vi "MetaData Channel.vi"(8 "error in (no error)":errorcluster, 11 "Node Ptr":T5 format="%.0x") -> (0 "error out":errorcluster)   [LabVIEW 2020, in "Instrument Addon System Explorer.lvlib"]
uses:
  Instrument Addon System Explorer.lvlib
  <vilib>/NI VeriStand/Custom Device API/Custom Device API.lvlib
  Addon Shared/Instrument Addon Shared.lvlib
  Addon Shared/Types/FG Control.ctl
  Addon Shared/SubVIs/Constants.vi
  APIs/Scripting API/Instrument Addon Scripting API.lvlib
  <vilib>/NI VeriStand/Custom Device API/Custom Device Item Ref.ctl
  Addon Shared/Types/Protocol Data Type.ctl
  Addon Shared/Types/Metadata Channel Type.ctl
  Addon Shared/Types/Type Cast Type.ctl
  Addon Shared/Types/Endian.ctl
panel:
  in  "Delimiter":string=","
  in  "Reset":bool
  in  "Create":bool
  in  "Elements":u32
  in  "Units":string
  in  "Default Value":dbl
  out "Channel Type (Tab)":enum32{"List", "Format", "Type Cast"}(tab)
  in  "Remove":bool
  in  "Add":bool
  in  "Enumerated List":i32(listbox)
  in  "Test Value":dbl
  in  "Format String":string="%.3g"
  out "Validated String":string
  in  "Endian":T1=enum."Little"
  in  "Type":T2
  in  "Channel Type":T3
  out "Data Type":T4
  in  "Header 2":cluster{"Section Name":string}={"Section Name"="MetaData Format Settings"}
  in  "SHDocVw.IWebBrowser":refnum<k7>(container)
  in  "Header":cluster{"Section Name":string}={"Section Name"="MetaData Settings"}
  in  "Description":string
  in  "Name":string
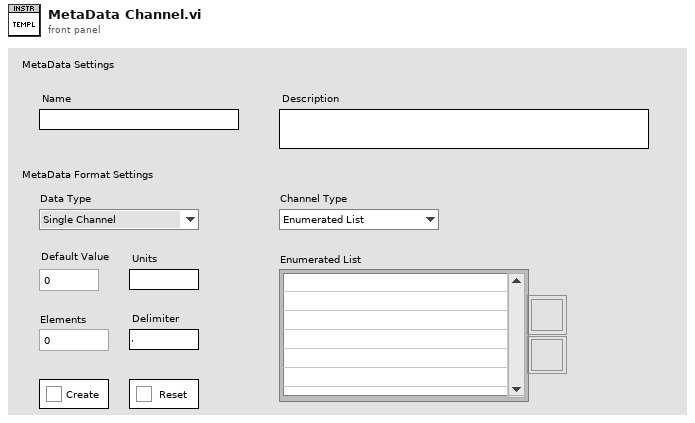
[diagram p1: front panel]
types:
  T1 = typedef "Instrument Addon Shared.lvlib/Endian.ctl" = enum16{"Native", "Little", "Big"}
  T2 = typedef "Instrument Addon Shared.lvlib/Type Cast Type.ctl" = enum16{"DBL", "SGL", "U64", "U32", "U16", "U8", "I64", "I32", "I16", "I8"}
  T3 = typedef "Instrument Addon Shared.lvlib/Metadata Channel Type.ctl" = enum16{"Enumerated List", "Format", "Type Cast"}
  T4 = typedef "Instrument Addon Shared.lvlib/Protocol Data Type.ctl" = enum16{"Single Channel", "Array"}
  T5 = typedef "Custom Device API.lvlib/Custom Device Item Ref.ctl" = u64
  T6 = typedef "Instrument Addon Shared.lvlib/FG Control.ctl" = enum16{"Get", "Set"}
  T7 = typedef "Custom Device API.lvlib/Custom Device Item Info.ctl" = cluster{"Name":string, "Is Channel":bool, "GUID":string, "Is Waveform":bool}
  T8 = typedef "Instrument Addon Shared.lvlib/MetaData Parameters.ctl" = cluster{"Data Type":T4, "Channel Type":T3, "List":string[], "Format String":string, "Type":T2, "Delimiter":string, "Endian":T1}
  T9 = typedef "Custom Device API.lvlib/Custom Device Channel.ctl" = cluster{"Type":T10, "Units":string, "Default Value":dbl, "Faultable":bool, "Scalable":bool}
  T10 = typedef "Custom Device API.lvlib/Custom Device Channel Type.ctl" = enum16{"Input", "Output"}
  T11 = typedef "Custom Device API.lvlib/Custom Device Commands.ctl" = enum16{"Default", "Item renamed", "Shutdown", "Dynamic button pressed"}
  T12 = typedef "Instrument Addon Scripting API.lvlib/Array Element.ctl" = cluster{"Name":string, "Default Value":dbl, "Units":string}
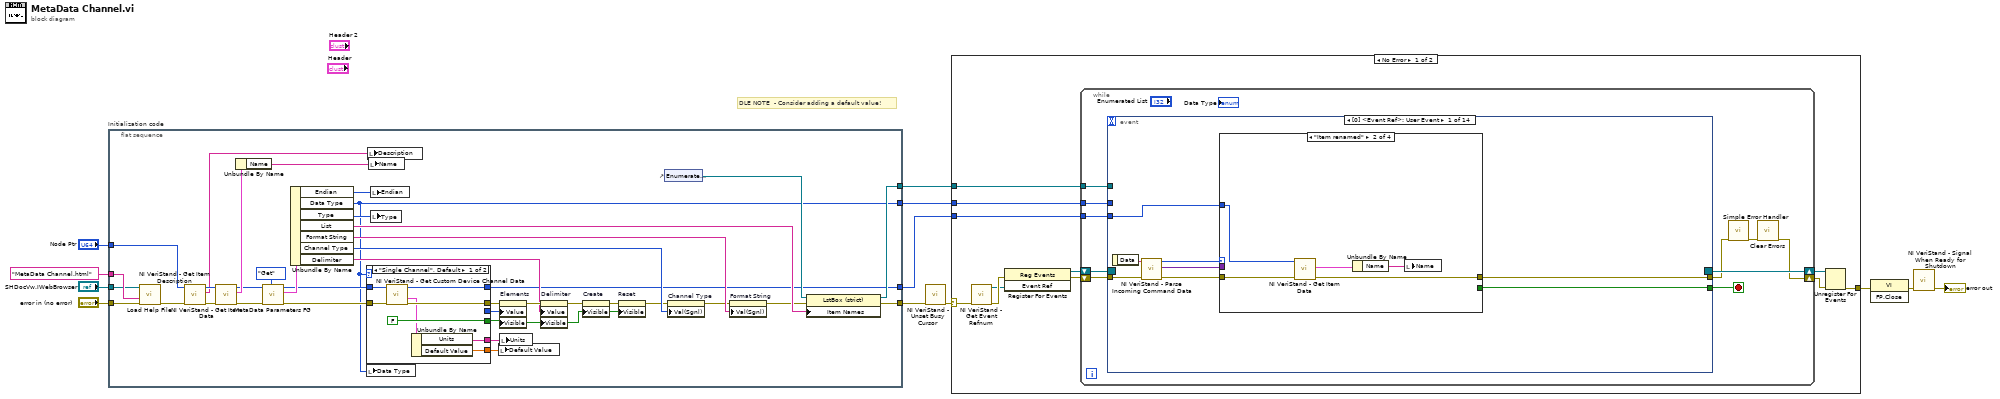
[diagram p0: block diagram]
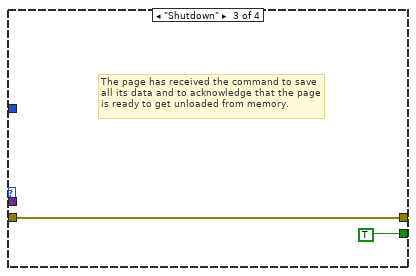
[diagram p3: hidden frame]
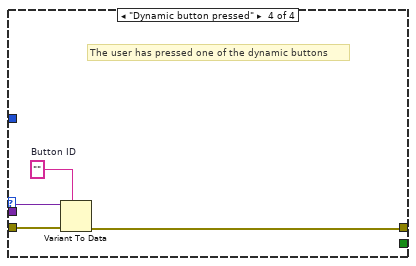
[diagram p4: hidden frame]
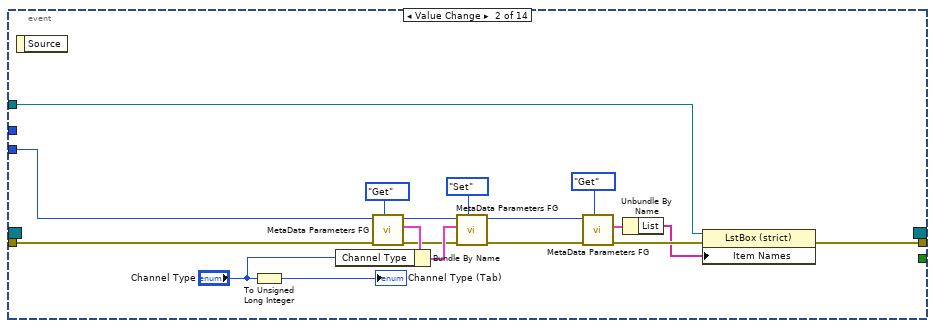
[diagram p5: hidden frame]
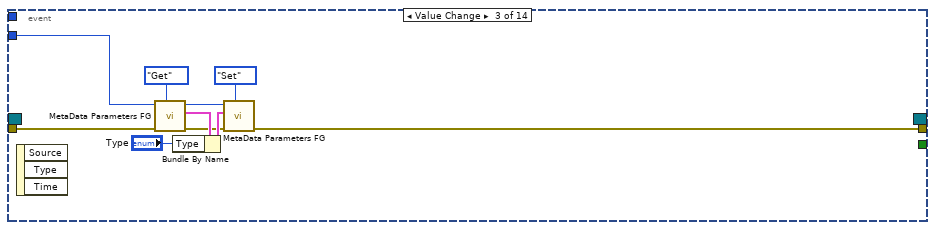
[diagram p6: hidden frame]
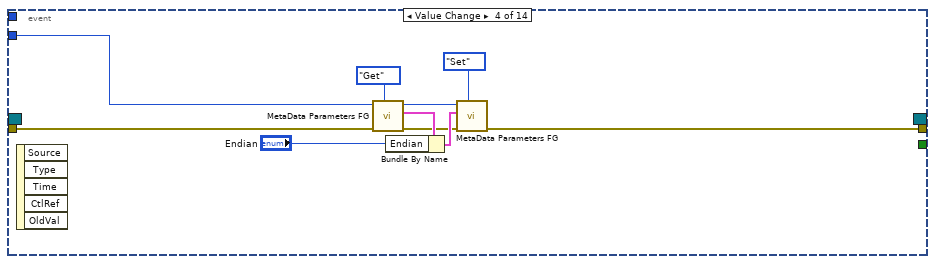
[diagram p7: hidden frame]
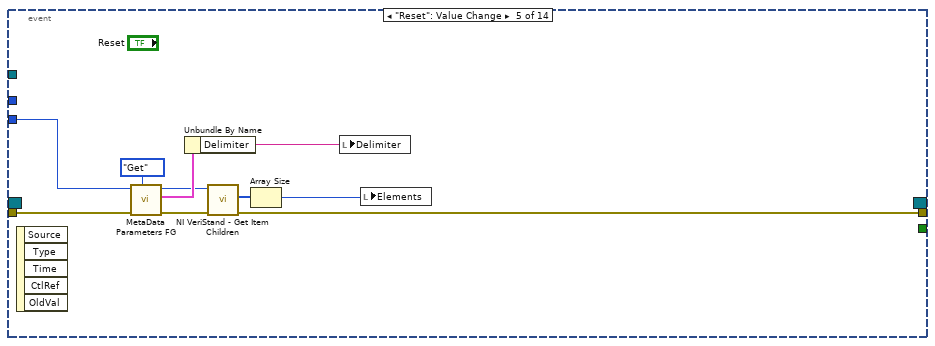
[diagram p8: hidden frame]
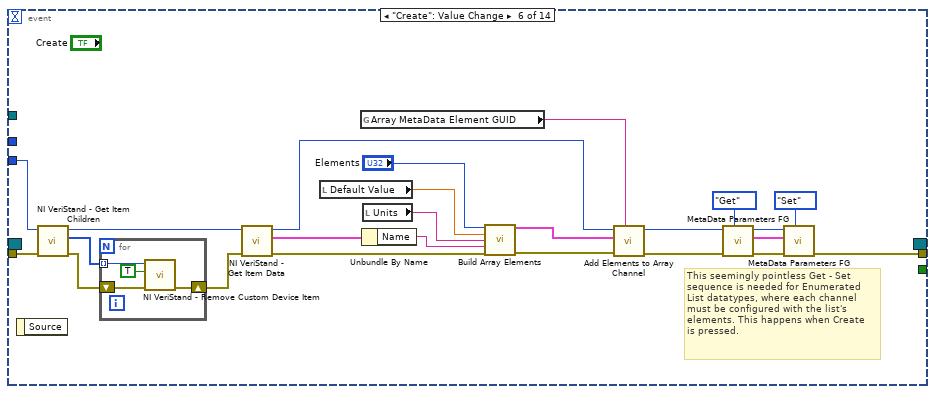
[diagram p9: hidden frame]
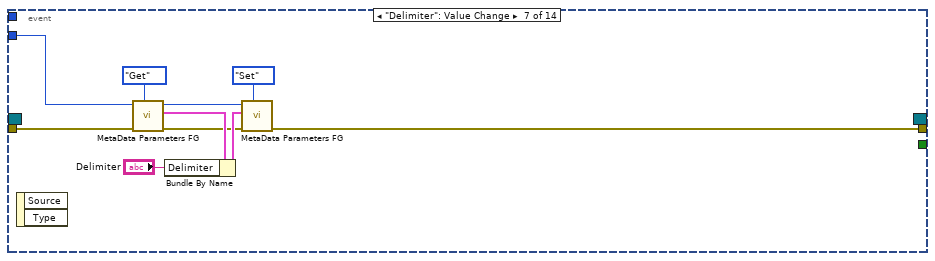
[diagram p10: hidden frame]
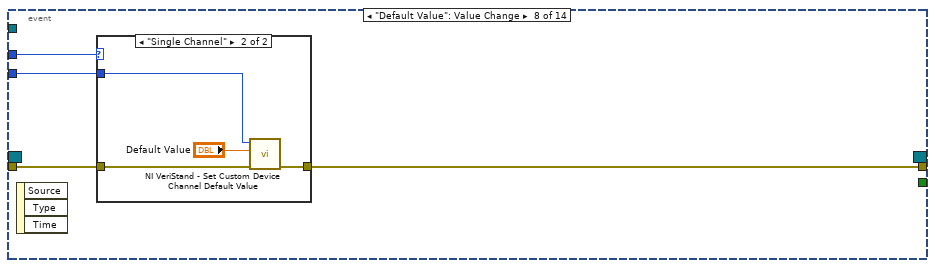
[diagram p11: hidden frame]
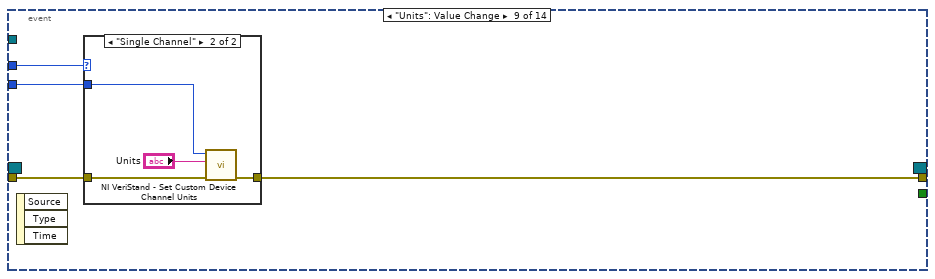
[diagram p13: hidden frame]
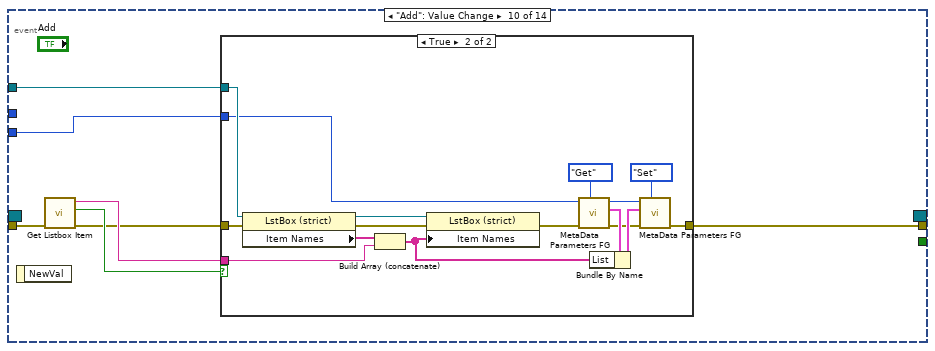
[diagram p15: hidden frame]
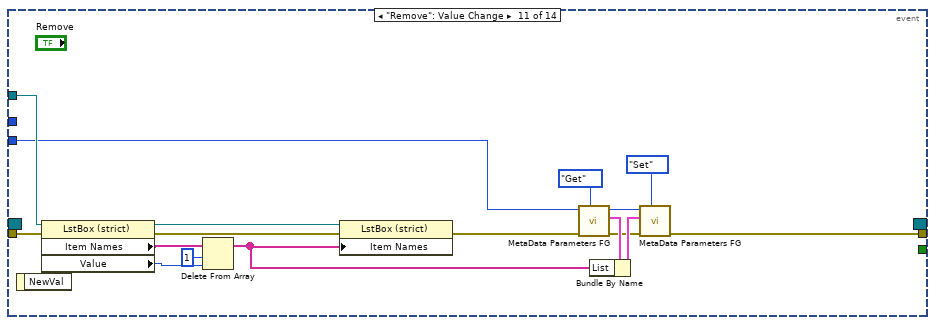
[diagram p17: hidden frame]
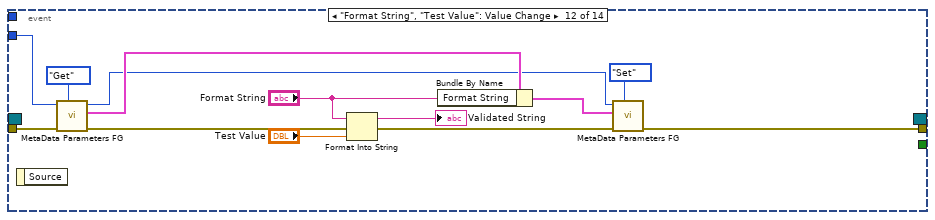
[diagram p18: hidden frame]
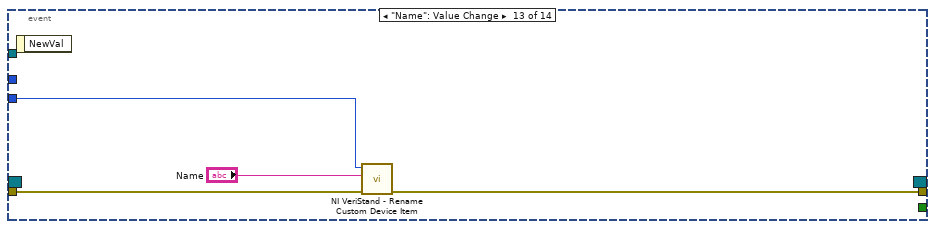
[diagram p19: hidden frame]
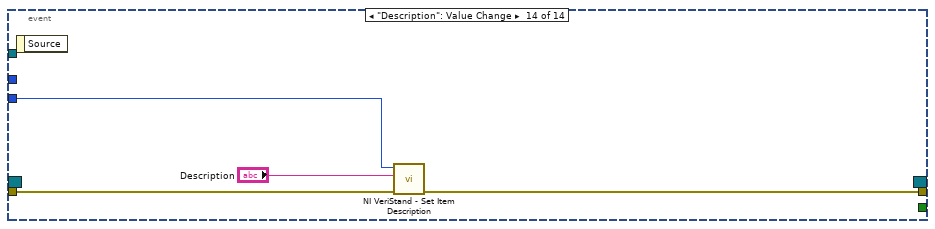
[diagram p20: hidden frame]
diagram:
  # "DLE NOTE  - Consider adding a default value!"
  n1 = flat-sequence "Initialization code" {
    tunnel: "error in (no error)" -> [w45]
    tunnel: "Node Ptr" -> [w31]
    tunnel: [w35] -> w8
    tunnel: [w19] -> w2
    tunnel: "MetaData Channel.html" ("HTML File") -> [w44]
    tunnel: "SHDocVw.IWebBrowser" -> [w43]
    tunnel: [w33] -> w3
    tunnel: [w16] -> w1
    frame #0 {
      n2 = call "Load Help File.vi"("error in (no error)"=w45, "HTML File to Load"=w44, "SHDocVw.IWebBrowser2"=w43) -> ("error out"=w32:errorcluster)  [unwired: 8 in]
      n3 = call <vilib>:"NI VeriStand - Get Item Description.vi"("error in (no error)"=w32, "Item Ref in"=w31) -> ("error out"=w48:errorcluster, "Description"=w49:string, "Item Ref out"=w50:T5)  [unwired: 7 out]
      n4 = call <vilib>:"NI VeriStand - Get Item Data.vi"("error in (no error)"=w48, "Item Ref in"=w50) -> ("error out"=w24:errorcluster, "Item Info"=w47:T7, "Item Ref out"=w23:T5)  [unwired: 7 out]
      n5 = Unbundle By Name(w47) -> ("Name"=w46:string)
      n6 = call "MetaData Parameters FG.vi"("Action"=FG_Control."Get", "error in (no error)"=w24, "Item Ref in"=w23) -> ("error out"=w22:errorcluster, "MetaData Parameters"=w41:T8, "Item Ref out"=w21:T5)  [unwired: 6 in]
      n7 = Unbundle By Name(w41) -> ("Endian"=w14:T1, "Data Type"=w16:T4, "Type"=w30:T2, "List"=w39:string[], "Format String"=w38:string, "Channel Type"=w40:T3, "Delimiter"=w25:string)
      n8 = local write "Data Type"(w16) -> ()
      n9 = case shown="\"Single Channel\", Default" w16 {
        tunnel: [FALSE TRUE] -> w13
        tunnel: w22 -> [w57 w62]
        tunnel: w21 -> [w56 w66]
        tunnel: [w55 w61] -> w20
        tunnel: [w54 w63] -> w19
        tunnel: [w52 ""] -> w18
        tunnel: [w51 0.0 ("Default Value")] -> w17
        tunnel: [_ w59] -> w15
        frame "Single Channel", Default {
          n10 = call <vilib>:"NI VeriStand - Get Custom Device Channel Data.vi"("error in (no error)"=w57, "Channel Ref in"=w56) -> ("error out"=w55:errorcluster, "Channel"=w53:T9, "Channel Ref out"=w54:T5)  [unwired: 4 in, 3 out]
          n11 = Unbundle By Name(w53) -> ("Units"=w52:string, "Default Value"=w51:dbl)
        }
        frame "Array" {
          n12 = call <vilib>:"NI VeriStand - Get Item Children.vi"("error in (no error)"=w62, "Item Ref in"=w66) -> ("error out"=w61:errorcluster, "Child Refs"=w60:T5[], "Item Ref out"=w63:T5)  [unwired: 6 in, 1 out]
          n13 = Array Size(array=w60) -> (size(s)=w59:i32)
        }
      }
      n14 = local write "Description"(w49) -> ()
      n15 = local write "Name"(w46) -> ()
      n16 = local write "Endian"(w14) -> ()
      n17 = local write "Type"(w30) -> ()
      n18 = local write "Default Value"(w17) -> ()
      n19 = property on="Elements" class="DigNum (strict)"(error in=w20, "Value"=w15, "Visible"=w13) -> (error out=w27:errorcluster)  [unwired: 1 in, 1 out]
      n20 = local write "Units"(w18) -> ()
      n21 = property on="Delimiter" class="Str"(error in=w27, "Value"=w25, "Visible"=w13) -> (error out=w28:errorcluster)  [unwired: 1 in, 1 out]
      n22 = property on="Create" class="Bool"(error in=w28, "Visible"=w13) -> (error out=w29:errorcluster)  [unwired: 1 in, 1 out]
      n23 = property on="Reset" class="Bool"(error in=w29, "Visible"=w13) -> (error out=w26:errorcluster)  [unwired: 1 in, 1 out]
      n24 = control-ref of="Enumerated List"() -> (w34:refnum<vi>)
      n25 = property on="Channel Type" class="Enum (strict)"(error in=w26, "Val(Sgnl)"=w40) -> (error out=w37:errorcluster)  [unwired: 1 in, 1 out]
      n26 = property on="Format String" class="Str"(error in=w37, "Val(Sgnl)"=w38) -> (error out=w36:errorcluster)  [unwired: 1 in, 1 out]
      n27 = property class="LstBox (strict)"(reference=w34, error in=w36, "Item Names"=w39) -> (reference out=w33:refnum<vi>, error out=w35:errorcluster)
    }
  }
  n28 = call <vilib>:"NI VeriStand - Unset Busy Cursor.vi"("error in (no error)"=w8) -> ("error out"=w7:errorcluster)  [unwired: 10 out]
  n29 = case shown="No Error" w7 {
    selector: w7 -> [w70 w277]
    tunnel: [w75 w275] -> w12
    tunnel: w2 -> [w71 _]
    tunnel: w3 -> [w69 _]
    tunnel: w1 -> [w68 _]
    frame No Error {
      n30 = call <vilib>:"NI VeriStand - Get Event Refnum.vi"("error in (no error)"=w70) -> ("error out"=w78:errorcluster, "Event Ref"=w74:refnum<user-event>)  [unwired: 9 out]
      n31 = register-events(error in=w78, w74) -> (reference out=w72:refnum<event-registration>, error out=w73:errorcluster)  [unwired: 1 in]
      n32 = while {
        tunnel: w71 -> [w84]
        shift-right: [w81] -> w76
        shift-left: w73 -> [w87]
        shift-right: [w88] -> w77
        shift-left: w72 -> [w86]
        tunnel: w69 -> [w80]
        tunnel: w68 -> [w79]
        stop <- w85 stop-if-true
        n33 = event shown="[0] <Event Ref>: User Event" {
          selector: w86 -> [_ _ _ _ _ _ _ _ _ _ _ _ _ _]
          dyn-events: [_ _ _ _ _ _ _ _ _ _ _ _ _ _] -> w88
          timeout: _ -> [_ _ _ _ _ _ _ _ _ _ _ _ _ _]
          tunnel: w87 -> [w96 w120 w131 w141 w154 w176 w187 w198 w207 w214 w250 w262 w270 w273]
          tunnel: [w92 _ _ _ _ _ _ _ _ _ _ _ _ _] -> w85
          tunnel: [w91 w109 w127 w138 w148 w167 w185 w197 w206 w218 w239 w263 w269 w272] -> w83
          tunnel: w84 -> [w90 w119 w130 w140 w153 w179 w186 w196 w205 w217 w237 w260 w268 w274]
          tunnel: w80 -> [_ w111 _ _ _ _ _ _ _ w219 w253 _ _ _]
          tunnel: w79 -> [_ _ _ _ _ _ _ w195 w204 _ _ _ _ _]
          event User Event {
            n34 = event-data() -> ("Data"=w95:string)  [unwired: 1 out]
            n35 = call <vilib>:"NI VeriStand - Parse Incoming Command Data.vi"("error in (no error)"=w96, "Incoming data"=w95) -> ("error out"=w94:errorcluster, "Outgoing data"=w89:variant, "Action"=w93:T11)  [unwired: 7 out]
            n36 = case shown="\"Item renamed\"" w93 {
              tunnel: w94 -> [w97 w102 w103 w108]
              tunnel: [_ _ TRUE _] -> w92
              tunnel: [w97 w99 w103 w105] -> w91
              tunnel: w90 -> [_ w101 _ _]
              tunnel: w89 -> [_ _ _ w107]
              frame "Default", Default {
              }
              frame "Item renamed" {
                n37 = call <vilib>:"NI VeriStand - Get Item Data.vi"("error in (no error)"=w102, "Item Ref in"=w101) -> ("error out"=w99:errorcluster, "Item Info"=w100:T7)  [unwired: 8 out]
                n38 = Unbundle By Name(w100) -> ("Name"=w98:string)
                n39 = local write "Name"(w98) -> ()
              }
              frame "Shutdown" {
                # "The page has received the command to save all its data and to acknowledge that the page is ready to get unloaded from memory."
              }
              frame "Dynamic button pressed" {
                w106 = ""  # Button ID
                # "The user has pressed one of the dynamic buttons"
                n40 = Variant To Data(error in=w108, type=w106, Variant=w107) -> (error out=w105:errorcluster)  [unwired: 1 out]
              }
            }
          }
          event Value Change {
            n41 = event-data() -> ()  [unwired: 2 out]
            n42 = To Unsigned Long Integer(number="Channel Type") -> (unsigned 32bit integer=→"Channel Type (Tab)":u32)
            n43 = call "MetaData Parameters FG.vi"("Action"=FG_Control."Get", "error in (no error)"=w120, "Item Ref in"=w119) -> ("error out"=w118:errorcluster, "MetaData Parameters"=w124:T8, "Item Ref out"=w122:T5)  [unwired: 6 in]
            n44 = Bundle By Name(cluster=w124, "Channel Type"="Channel Type") -> (w123:T8)
            n45 = call "MetaData Parameters FG.vi"("Action"=FG_Control."Set", "error in (no error)"=w118, "MetaData Parameters"=w123, "Item Ref in"=w122) -> ("error out"=w113:errorcluster, "Item Ref out"=w112:T5)  [unwired: 5 in, 1 out]
            n46 = call "MetaData Parameters FG.vi"("Action"=FG_Control."Get", "error in (no error)"=w113, "Item Ref in"=w112) -> ("error out"=w115:errorcluster, "MetaData Parameters"=w116:T8)  [unwired: 6 in, 1 out]
            n47 = Unbundle By Name(w116) -> ("List"=w114:string[])
            n48 = property class="LstBox (strict)"(reference=w111, error in=w115, "Item Names"=w114) -> (error out=w109:errorcluster)  [unwired: 1 out]
          }
          event Value Change {
            n49 = event-data() -> ()  [unwired: 4 out]
            n50 = call "MetaData Parameters FG.vi"("Action"=FG_Control."Get", "error in (no error)"=w131, "Item Ref in"=w130) -> ("error out"=w129:errorcluster, "MetaData Parameters"=w135:T8, "Item Ref out"=w133:T5)  [unwired: 6 in]
            n51 = Bundle By Name(cluster=w135, "Type"="Type") -> (w134:T8)
            n52 = call "MetaData Parameters FG.vi"("Action"=FG_Control."Set", "error in (no error)"=w129, "MetaData Parameters"=w134, "Item Ref in"=w133) -> ("error out"=w127:errorcluster)  [unwired: 5 in, 2 out]
          }
          event Value Change {
            n53 = event-data() -> ()  [unwired: 6 out]
            n54 = call "MetaData Parameters FG.vi"("Action"=FG_Control."Get", "error in (no error)"=w141, "Item Ref in"=w140) -> ("error out"=w139:errorcluster, "MetaData Parameters"=w145:T8, "Item Ref out"=w143:T5)  [unwired: 6 in]
            n55 = Bundle By Name(cluster=w145, "Endian"="Endian") -> (w144:T8)
            n56 = call "MetaData Parameters FG.vi"("Action"=FG_Control."Set", "error in (no error)"=w139, "MetaData Parameters"=w144, "Item Ref in"=w143) -> ("error out"=w138:errorcluster)  [unwired: 5 in, 2 out]
          }
          event "Reset": Value Change {
            n57 = event-data() -> ()  [unwired: 6 out]
            n58 = call "MetaData Parameters FG.vi"("Action"=FG_Control."Get", "error in (no error)"=w154, "Item Ref in"=w153) -> ("error out"=w149:errorcluster, "MetaData Parameters"=w156:T8, "Item Ref out"=w150:T5)  [unwired: 6 in]
            n59 = Unbundle By Name(w156) -> ("Delimiter"=w152:string)
            n60 = call <vilib>:"NI VeriStand - Get Item Children.vi"("error in (no error)"=w149, "Item Ref in"=w150) -> ("error out"=w148:errorcluster, "Child Refs"=w151:T5[])  [unwired: 6 in, 2 out]
            n61 = Array Size(array=w151) -> (size(s)=w147:i32)
            n62 = local write "Delimiter"(w152) -> ()
            n63 = local write "Elements"(w147) -> ()
          }
          event "Create": Value Change {
            # "This seemingly pointless Get - Set\nsequence is needed for Enumerated\nList datatypes, where each channel\nmust be configured with the list's\nelements. This happens when Create\nis pressed."
            n64 = event-data() -> ()  [unwired: 2 out]
            n65 = call <vilib>:"NI VeriStand - Get Item Children.vi"("error in (no error)"=w176, "Item Ref in"=w179) -> ("error out"=w173:errorcluster, "Child Refs"=w174:T5[], "Item Ref out"=w177:T5)  [unwired: 6 in, 1 out]
            n66 = for {
              shift-right: [w183] -> w175
              shift-left: w173 -> [w181]
              tunnel: w174 -> [w182] mode=indexing
              n67 = call <vilib>:"NI VeriStand - Remove Custom Device Item.vi"("error in (no error)"=w181, "Force Delete (F)"=TRUE, "Item Ref in"=w182) -> ("error out"=w183:errorcluster)  [unwired: 7 in, 1 out]
            }
            n68 = call <vilib>:"NI VeriStand - Get Item Data.vi"("error in (no error)"=w175, "Item Ref in"=w177) -> ("error out"=w178:errorcluster, "Item Info"=w180:T7, "Item Ref out"=w162:T5)  [unwired: 7 out]
            n69 = local read "Default Value"() -> (w164:dbl)
            n70 = global read "Constants.vi" "Array MetaData Element GUID"() -> (w157:string)
            n71 = Unbundle By Name(w180) -> ("Name"=w166:string)
            n72 = local read "Units"() -> (w165:string)
            n73 = call "Build Array Elements.vi"("Elements"="Elements", "Default Value"=w164, "Units"=w165, "Name"=w166, "error in (no error)"=w178) -> ("Array"=w161:T12[], "error out"=w160:errorcluster)  [unwired: 9 in]
            n74 = call "Add Elements to Array Channel.vi"("array element GUID"=w157, "error in (no error)"=w160, "array elements"=w161, "array refnum in"=w162) -> ("error out"=w159:errorcluster, "array refnum out"=w158:T5)  [unwired: 5 in, 1 out]
            n75 = call "MetaData Parameters FG.vi"("Action"=FG_Control."Get", "error in (no error)"=w159, "Item Ref in"=w158) -> ("error out"=w169:errorcluster, "MetaData Parameters"=w168:T8, "Item Ref out"=w171:T5)  [unwired: 6 in]
            n76 = call "MetaData Parameters FG.vi"("Action"=FG_Control."Set", "error in (no error)"=w169, "MetaData Parameters"=w168, "Item Ref in"=w171) -> ("error out"=w167:errorcluster)  [unwired: 5 in, 2 out]
          }
          event "Delimiter": Value Change {
            n77 = event-data() -> ()  [unwired: 3 out]
            n78 = call "MetaData Parameters FG.vi"("Action"=FG_Control."Get", "error in (no error)"=w187, "Item Ref in"=w186) -> ("error out"=w190:errorcluster, "MetaData Parameters"=w194:T8, "Item Ref out"=w192:T5)  [unwired: 6 in]
            n79 = Bundle By Name(cluster=w194, "Delimiter"="Delimiter") -> (w193:T8)
            n80 = call "MetaData Parameters FG.vi"("Action"=FG_Control."Set", "error in (no error)"=w190, "MetaData Parameters"=w193, "Item Ref in"=w192) -> ("error out"=w185:errorcluster)  [unwired: 5 in, 2 out]
          }
          event "Default Value": Value Change {
            n81 = event-data() -> ()  [unwired: 4 out]
            n82 = case shown="\"Single Channel\"" w195 {
              tunnel: w198 -> [w199 w203]
              tunnel: [w199 w202] -> w197
              tunnel: w196 -> [_ w201]
              frame "Array" {
              }
              frame "Single Channel" {
                n83 = call <vilib>:"NI VeriStand - Set Custom Device Channel Default Value.vi"("error in (no error)"=w203, "Default Value"="Default Value", "Channel Ref in"=w201) -> ("error out"=w202:errorcluster)  [unwired: 7 in, 1 out]
              }
            }
          }
          event "Units": Value Change {
            n84 = event-data() -> ()  [unwired: 4 out]
            n85 = case shown="\"Single Channel\"" w204 {
              tunnel: w207 -> [w208 w212]
              tunnel: [w208 w211] -> w206
              tunnel: w205 -> [_ w210]
              frame "Array" {
              }
              frame "Single Channel" {
                n86 = call <vilib>:"NI VeriStand - Set Custom Device Channel Units.vi"("error in (no error)"=w212, "Units"="Units", "Channel Ref in"=w210) -> ("error out"=w211:errorcluster)  [unwired: 7 in, 1 out]
              }
            }
          }
          event "Add": Value Change {
            n87 = event-data() -> ()  [unwired: 2 out]
            n88 = call "Get Listbox Item.vi"("error in (no error)"=w214) -> ("error out"=w213:errorcluster, "OK?"=w215:bool, "Item out"=w216:string)  [unwired: 8 in]
            n89 = case shown="True" w215 {
              tunnel: w219 -> [_ w236]
              tunnel: w213 -> [w220 w235]
              tunnel: w216 -> [_ w231]
              tunnel: [w220 w222] -> w218
              tunnel: w217 -> [_ w224]
              frame False {
              }
              frame True {
                n90 = property class="LstBox (strict)"(reference=w236, error in=w235) -> (reference out=w234:refnum<vi>, error out=w233:errorcluster, "Item Names"=w232:string[])
                n91 = Build Array (concatenate)(w232, w231) -> (w221:string[])
                n92 = property class="LstBox (strict)"(reference=w234, error in=w233, "Item Names"=w221) -> (error out=w223:errorcluster)  [unwired: 1 out]
                n93 = call "MetaData Parameters FG.vi"("Action"=FG_Control."Get", "error in (no error)"=w223, "Item Ref in"=w224) -> ("error out"=w225:errorcluster, "MetaData Parameters"=w229:T8, "Item Ref out"=w227:T5)  [unwired: 6 in]
                n94 = Bundle By Name(cluster=w229, "List"=w221) -> (w228:T8)
                n95 = call "MetaData Parameters FG.vi"("Action"=FG_Control."Set", "error in (no error)"=w225, "MetaData Parameters"=w228, "Item Ref in"=w227) -> ("error out"=w222:errorcluster)  [unwired: 5 in, 2 out]
              }
            }
          }
          event "Remove": Value Change {
            n96 = event-data() -> ()  [unwired: 2 out]
            n97 = property class="LstBox (strict)"(reference=w253, error in=w250) -> (reference out=w252:refnum<vi>, error out=w251:errorcluster, "Item Names"=w249:string[], "Value"=w248:i32)
            n98 = Delete From Array(array=w249, length=1, index=w248) -> (array with subset deleted=w238:string[])  [unwired: 1 out]
            n99 = property class="LstBox (strict)"(reference=w252, error in=w251, "Item Names"=w238) -> (error out=w240:errorcluster)  [unwired: 1 out]
            n100 = call "MetaData Parameters FG.vi"("Action"=FG_Control."Get", "error in (no error)"=w240, "Item Ref in"=w237) -> ("error out"=w241:errorcluster, "MetaData Parameters"=w245:T8, "Item Ref out"=w243:T5)  [unwired: 6 in]
            n101 = Bundle By Name(cluster=w245, "List"=w238) -> (w244:T8)
            n102 = call "MetaData Parameters FG.vi"("Action"=FG_Control."Set", "error in (no error)"=w241, "MetaData Parameters"=w244, "Item Ref in"=w243) -> ("error out"=w239:errorcluster)  [unwired: 5 in, 2 out]
          }
          event "Format String", "Test Value": Value Change {
            n103 = event-data() -> ()  [unwired: 2 out]
            n104 = call "MetaData Parameters FG.vi"("Action"=FG_Control."Get", "error in (no error)"=w262, "Item Ref in"=w260) -> ("error out"=w261:errorcluster, "MetaData Parameters"=w258:T8, "Item Ref out"=w255:T5)  [unwired: 6 in]
            n105 = Format Into String(format string="Format String", error in=w261, "Test Value") -> (resulting string=→"Validated String":string, error out=w264:errorcluster)  [unwired: 1 in]
            n106 = Bundle By Name(cluster=w258, "Format String"="Format String") -> (w256:T8)
            n107 = call "MetaData Parameters FG.vi"("Action"=FG_Control."Set", "error in (no error)"=w264, "MetaData Parameters"=w256, "Item Ref in"=w255) -> ("error out"=w263:errorcluster)  [unwired: 5 in, 2 out]
          }
          event "Name": Value Change {
            n108 = event-data() -> ()  [unwired: 2 out]
            n109 = call <vilib>:"NI VeriStand - Rename Custom Device Item.vi"("error in (no error)"=w270, "New Name"="Name", "Item Ref in"=w268) -> ("error out"=w269:errorcluster)  [unwired: 1 in, 7 out]
          }
          event "Description": Value Change {
            n110 = event-data() -> ()  [unwired: 2 out]
            n111 = call <vilib>:"NI VeriStand - Set Item Description.vi"("error in (no error)"=w273, "Description"="Description", "Item Ref in"=w274) -> ("error out"=w272:errorcluster)  [unwired: 8 out]
          }
        }
        n112 = call <vilib>:"Simple Error Handler.vi"("error in (no error)"=w83) -> ("error out"=w82:errorcluster)  [unwired: 1 in, 7 out]
        n113 = call <vilib>:"Clear Errors.vi"("error in (no error)"=w82) -> ("error out"=w81:errorcluster)  [unwired: 1 in, 5 out]
      }
      n114 = Unregister For Events(event registration refnum=w77, error in=w76) -> (error out=w75:errorcluster)
    }
    frame Error {
      n115 = call <vilib>:"Simple Error Handler.vi"("error in (no error)"=w277) -> ("error out"=w276:errorcluster)  [unwired: 1 in, 7 out]
      n116 = call <vilib>:"Clear Errors.vi"("error in (no error)"=w276) -> ("error out"=w275:errorcluster)  [unwired: 1 in, 5 out]
    }
  }
  n117 = invoke class="VI" method="FP.Close"(error in=w12) -> (error out=w11:errorcluster)  [unwired: 2 in, 2 out]
  n118 = call <vilib>:"NI VeriStand - Signal When Ready for Shutdown.vi"("error in (no error)"=w11) -> ("error out"=→"error out":errorcluster)  [unwired: 10 out]
